vi "Next.vi"(8 "error in (no error)":errorcluster, 11 "LUnit Test Suite In":refnum<class "LUnit Test Suite.lvclass">) -> (0 "error out":errorcluster, 2 "Next Runnable":string, 3 "LUnit Test Suite Out":refnum<class "LUnit Test Suite.lvclass">)   [LabVIEW 2020, in "LUnit Test Suite.lvclass"]
doc: "Get next active test in suite. This works recursively for nested suites."
uses:
  LUnit Test Suite.lvclass
  LUnit Test Suite.lvclass/LUnit Test Suite.ctl
  Runnable.lvclass
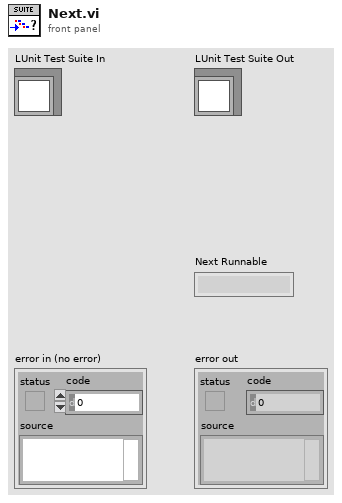
[diagram p1: front panel]
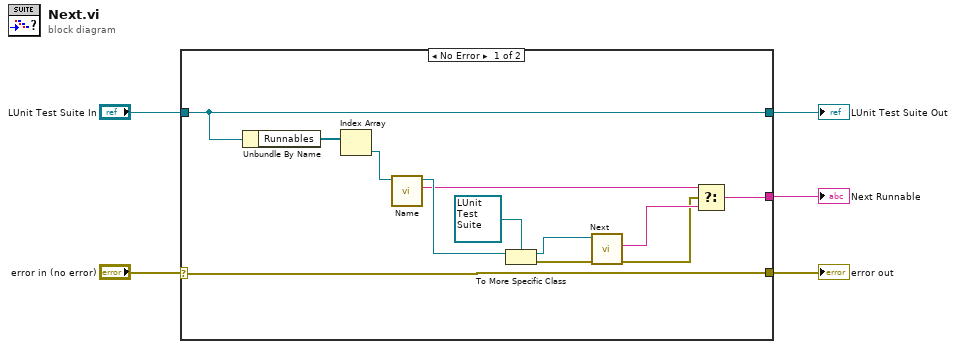
[diagram p0: block diagram]
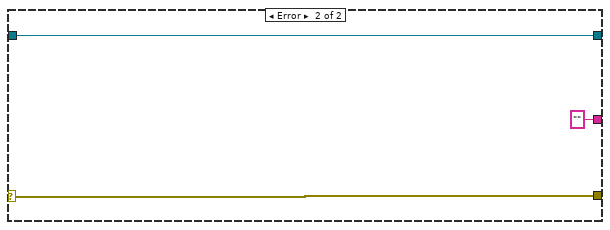
[diagram p2: hidden frame]
diagram:
  n1 = case shown="No Error" "error in (no error)" {
    selector: "error in (no error)" -> [w6 w19]
    tunnel: "LUnit Test Suite In" -> [w7 w20]
    tunnel: [w17 "" ("Next Runnable")] -> w4
    tunnel: [w7 w20] -> w2
    tunnel: [w6 w19] -> w1
    frame No Error {
      n2 = Unbundle By Name(w7) -> ("Runnables"=w11:refnum<class "Runnable.lvclass">[])
      n3 = Index Array(array=w11) -> (element=w10:refnum<class "Runnable.lvclass">)  [unwired: 1 in]
      n4 = call-dynamic "Name.vi"("Runnable in"=w10) -> ("Name"=w8:string, "Runnable out"=w9:refnum<class "Runnable.lvclass">)  [unwired: 8 in, 1 out]
      n5 = To More Specific Class(target class=refnum<class "LUnit Test Suite.lvclass"> refnum ("LUnit Test Suite Out"), reference=w9) -> (specific class reference=w16:refnum<class "LUnit Test Suite.lvclass">, error out=w14:errorcluster)  [unwired: 1 in]
      n6 = call "Next.vi"("error in (no error)"=w14, "LUnit Test Suite In"=w16) -> ("error out"=w12:errorcluster, "Next Runnable"=w13:string)  [unwired: 7 in, 1 out]
      n7 = Select(t=w8, s=w12, f=w13) -> (s? t:f=w17:string)
    }
    frame Error {
    }
  }
  "error out" <- w1
  "LUnit Test Suite Out" <- w2
  "Next Runnable" <- w4
